vi "Update.vi"(8 "error in":errorcluster, 10 "object ref in":T1, 11 "Multi Column Listbox in":refnum<class "Multi Column Listbox.lvclass">) -> (0 "error out":errorcluster, 2 "object ref out":T1, 3 "Multi Column Listbox out":refnum<class "Multi Column Listbox.lvclass">)   [LabVIEW 2014, in "Table Manager.lvlib" / "Multi Column Listbox.lvclass"]
doc: "Updates the strings displayed in the MCLB."
uses:
  Multi Column Listbox.lvclass
  Table Manager/object ref.ctl
  Configuration Editor/Classes/Engine Parent/Engine Parent Editor Node.lvclass
  Configuration Editor/Classes/Module editor node/module editor node.lvclass
  Multi Column Listbox.lvclass/Multi Column Listbox.ctl
  Table Manager/Table Manager.lvclass/Table Manager.ctl
  Read Listbox.vi
  Table Manager/Read Index.vi
  Table Manager/Table Manager.lvclass
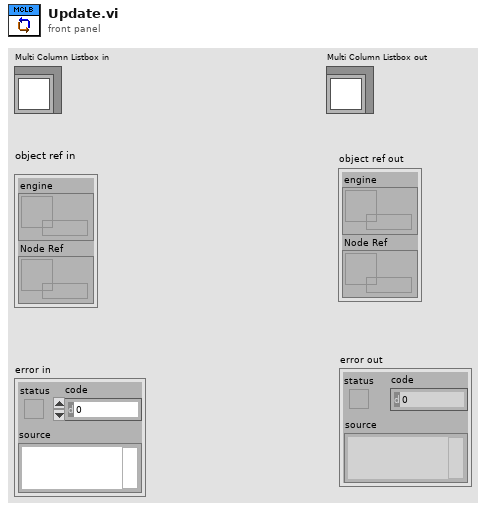
[diagram p1: front panel]
types:
  T1 = typedef "Table Manager.lvlib/Table Manager.lvclass/object ref.ctl" = cluster{"engine":refnum<data-value>, "Node Ref":refnum<data-value>}
  T2 = typedef "LVRowAndColumnTypeDef.ctl" = cluster{"Row":i32, "Column":i32}
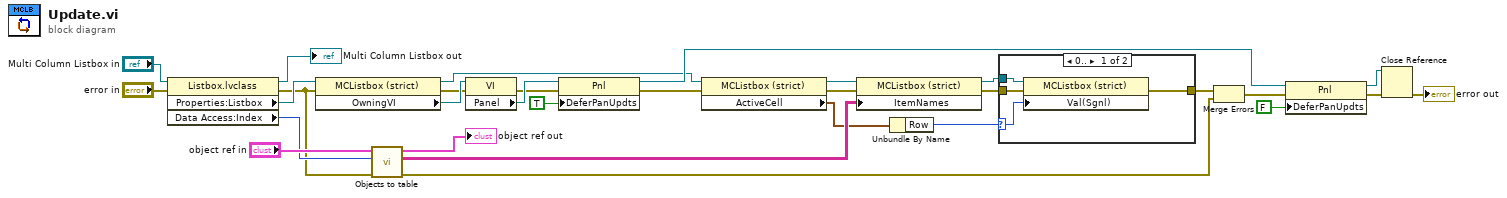
[diagram p0: block diagram]
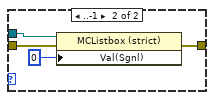
[diagram p2: hidden frame]
diagram:
  n1 = property class="Listbox.lvclass"(reference="Multi Column Listbox in", error in="error in") -> (reference out=→"Multi Column Listbox out":refnum<class "Multi Column Listbox.lvclass">, error out=w3:errorcluster, "Properties:Listbox"=w7:refnum<vi>, "Data Access:Index"=w8:i32)
  n2 = property class="MCListbox (strict)"(reference=w7, error in=w3) -> (reference out=w24:refnum<vi>, error out=w22:errorcluster, "OwningVI"=w23:refnum<vi>)
  n3 = call "Objects to table.vi"("error in (no error)"=w3, "Table Index"=w8, "object ref in"="object ref in") -> ("error out"=w11:errorcluster, "table"=w14:string[][], "object ref out"=→"object ref out":T1)  [unwired: 6 in]
  n4 = property class="VI"(reference=w23, error in=w22) -> (error out=w28:errorcluster, "Panel"=w29:refnum<vi>)  [unwired: 1 out]
  n5 = property class="Pnl"(reference=w29, error in=w28, "DeferPanUpdts"=TRUE ("Defer Panel Updates")) -> (reference out=w26:refnum<vi>, error out=w16:errorcluster)
  n6 = property class="MCListbox (strict)"(reference=w24, error in=w16) -> (reference out=w20:refnum<vi>, error out=w17:errorcluster, "ActiveCell"=w2:T2)
  n7 = property class="MCListbox (strict)"(reference=w20, error in=w17, "ItemNames"=w14) -> (reference out=w19:refnum<vi>, error out=w18:errorcluster)
  n8 = Unbundle By Name(w2) -> ("Row"=w1:i32)
  n9 = case shown="0.." w1 {
    selector: w1 -> [w31 _]
    tunnel: w19 -> [w34 w38]
    tunnel: w18 -> [w33 w37]
    tunnel: [w32 w36] -> w12
    frame 0.. {
      n10 = property class="MCListbox (strict)"(reference=w34, error in=w33, "Val(Sgnl)"=w31) -> (error out=w32:errorcluster)  [unwired: 1 out]
    }
    frame ..-1 {
      n11 = property class="MCListbox (strict)"(reference=w38, error in=w37, "Val(Sgnl)"=0 ("Value (Signaling)")) -> (error out=w36:errorcluster)  [unwired: 1 out]
    }
  }
  n12 = Merge Errors(w12, w11) -> (w10:errorcluster)
  n13 = property class="Pnl"(reference=w26, error in=w10, "DeferPanUpdts"=FALSE ("Defer Panel Updates")) -> (reference out=w21:refnum<vi>, error out=w25:errorcluster)
  n14 = Close Reference(reference=w21, error in (no error)=w25) -> (error out=→"error out":errorcluster)
